vi "Get Plot Visibility (WFGraph).vi"(8 "error in (no error)":errorcluster, 11 "WFGraph in":refnum<vi>) -> (0 "error out":errorcluster, 2 "Plot.Visible":bool[](array[boolean]))   [LabVIEW 2019, in "Instrument.Lockin.lvlib" / "Instrument UI.Lockin.lvclass"]
uses:
  Instrument UI.Lockin.lvclass
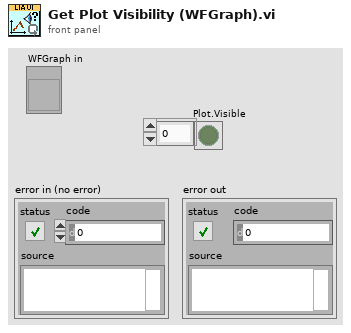
[diagram p1: front panel]
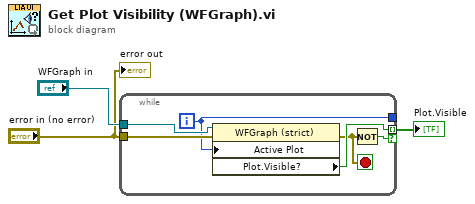
[diagram p0: block diagram]
diagram:
  n1 = while {
    tunnel: "WFGraph in" -> [w9]
    tunnel: [w4] -> _
    tunnel: [w8] -> w1 mode=indexing if=w6
    tunnel: "error in (no error)" -> [w5]
    i -> [w4]
    stop <- w7 stop-if-true
    n2 = property on="Property Node" class="WFGraph (strict)"(reference=w9, error in=w5, "Active Plot"=w4) -> (error out=w7:errorcluster, "Plot.Visible?"=w8:bool)  [unwired: 1 out]
    n3 = Not(x=w7) -> (.not. x?=w6:bool)
  }
  "Plot.Visible" <- w1
  "error out" <- "error in (no error)"
